vi "SC Close Project.vi"(8 "error in (no error)":errorcluster, 9 "project folder":path) -> (0 "error out":errorcluster, 1 "project path":path, 2 "closed?":bool)   [LabVIEW 2023]
doc: "Closes the open LabVIEW project in project folder (the one systemcore-deploy works on), before systemcore-deploy changes its files, and returns its path for SC Reopen Project. Without a folder, or when no open project is in it, closes LabVIEW's active project. closed? is false when there is no such project."
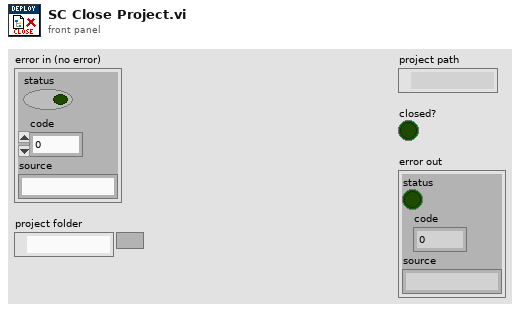
[diagram p1: front panel]
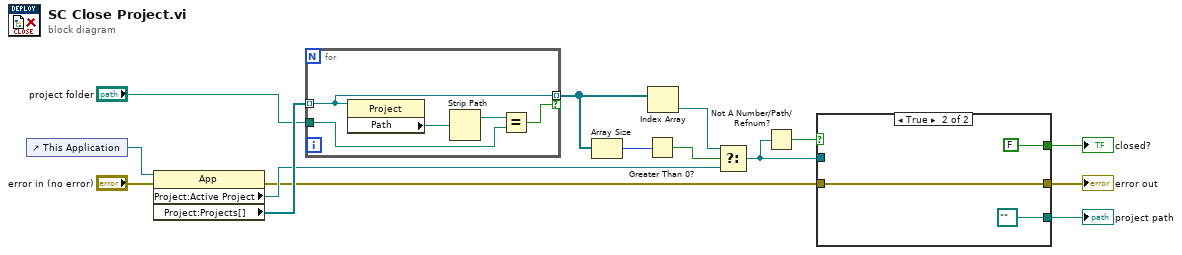
[diagram p0: block diagram]
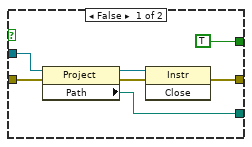
[diagram p2: hidden frame]
diagram:
  n1 = control-ref of="This Application"() -> (w15:refnum<vi>)
  n2 = property class="App"(reference=w15, error in="error in (no error)") -> (error out=w5:errorcluster, "Project:Active Project"=w7:refnum<vi>, "Project:Projects[]"=w13:refnum<vi>[])  [unwired: 1 out]
  n3 = for {
    tunnel: w13 -> [w16] mode=indexing
    tunnel: "project folder" -> [w18]
    tunnel: [w16] -> w10 mode=indexing if=w17
    n4 = property class="Project"(reference=w16) -> ("Path"=w20:path)  [unwired: 1 in, 2 out]
    n5 = Strip Path(path=w20) -> (stripped path=w19:path)  [unwired: 1 out]
    n6 = Equal?(x=w19, y=w18) -> (x = y?=w17:bool)
  }
  n7 = Array Size(array=w10) -> (size(s)=w11:i32)
  n8 = Greater Than 0?(x=w11) -> (x > 0?=w9:bool)
  n9 = Index Array(array=w10) -> (element=w8:refnum<vi>)  [unwired: 1 in]
  n10 = Select(t=w8, s=w9, f=w7) -> (s? t:f=w6:refnum<vi>)
  n11 = Not A Number/Path/Refnum?(number/path/refnum=w6) -> (NaN/Path/Refnum?=w1:bool)
  n12 = case shown="True" w1 {
    tunnel: w6 -> [w27 _]
    tunnel: w5 -> [w26 w30]
    tunnel: [w23 w30] -> w4
    tunnel: [w22 path ""] -> w3
    tunnel: [TRUE FALSE] -> w2
    frame False {
      n13 = property class="Project"(reference=w27, error in=w26) -> (reference out=w25:refnum<vi>, error out=w24:errorcluster, "Path"=w22:path)
      n14 = invoke class="Instr" method="Close"(reference=w25, error in=w24) -> (error out=w23:errorcluster)  [unwired: 1 in, 2 out]
    }
    frame True {
    }
  }
  "project path" <- w3
  "closed?" <- w2
  "error out" <- w4
